vi "Sub.vi"(5 "X":dbl, 7 "Gain":dbl, 11 "error in":errorcluster) -> (4 "Sum":dbl, 6 "Status":bool, 15 "error out":errorcluster)   [LabVIEW 2026]
doc: "Issue 136 subVI example, version 2: Y renamed Gain, Result renamed Sum, a new Status output."
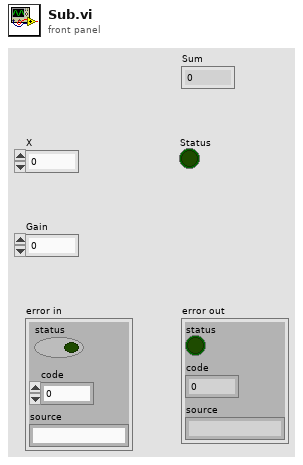
[diagram p1: front panel]
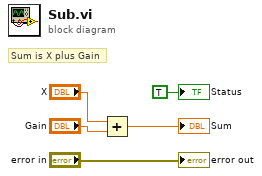
[diagram p0: block diagram]
diagram:
  # "Sum is X plus Gain"
  n1 = Add(x="X", y="Gain") -> (x+y=→"Sum":dbl)
  "Status" <- TRUE ("ok")
  "error out" <- "error in"
